vi "Start (App INI).vi"(7 "Splash Screen (Default)":refnum<class "Splash Screen.lvclass">, 8 "error in (no error)":errorcluster, 10 "INI Path (Default)":path) -> (0 "error out":errorcluster, 2 "MessageQ":refnum<class "MessageQ.lvclass">)   [LabVIEW 2020, in "Volatus.lvlib" / "Volatus Core.lvclass"]
uses:
  Volatus Core.lvclass
  MessageQ/MessageQ.lvclass
  Splash Screen/Splash Screen.lvclass
  Volatus Core.lvclass/Volatus Core.ctl
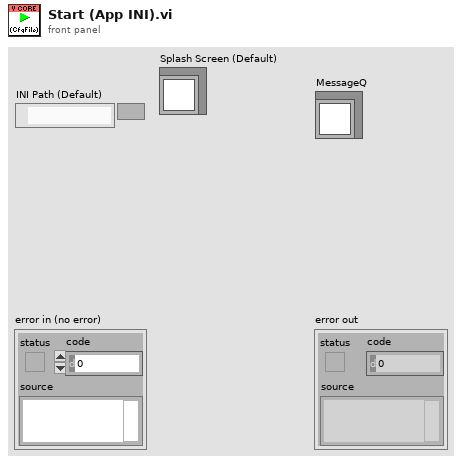
[diagram p1: front panel]
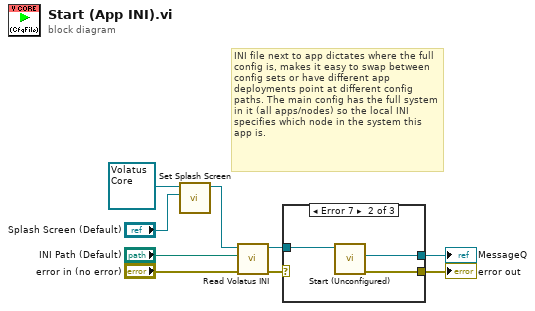
[diagram p0: block diagram]
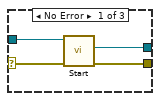
[diagram p2: hidden frame]
diagram:
  # "INI file next to app dictates where the full config is, makes it easy to swap between config sets or have different app deployments point at different config paths. The main config has the full system in it (all apps/nodes) so the local INI specifies which node in the system this app is."
  n1 = call "Set Splash Screen.vi"("Splash Screen"="Splash Screen (Default)", "Volatus Core in"=refnum<class "Volatus Core.lvclass"> refnum) -> ("Volatus Core out"=w1:refnum<class "Volatus Core.lvclass">)  [unwired: 8 in, 1 out]
  n2 = call "Read Volatus INI.vi"("error in (no error)"="error in (no error)", "INI Path (Default)"="INI Path (Default)", "Volatus Core in"=w1) -> ("error out"=w4:errorcluster, "Volatus Core out"=w5:refnum<class "Volatus Core.lvclass">)  [unwired: 7 in]
  n3 = case shown="Error 7" w4 {
    selector: w4 -> [w12 _ w17]
    tunnel: [w11 w15 w17] -> w7
    tunnel: [w10 w14 _] -> w8
    tunnel: w5 -> [w13 w16 _]
    frame No Error {
      n4 = call "Start.vi"("error in (no error)"=w12, "Volatus Core in"=w13) -> ("error out"=w11:errorcluster, "MessageQ"=w10:refnum<class "MessageQ.lvclass">)  [unwired: 8 in]
    }
    frame Error {
      n5 = call "Start (Unconfigured).vi"("Volatus Core in"=w16) -> ("error out"=w15:errorcluster, "MessageQ"=w14:refnum<class "MessageQ.lvclass">)  [unwired: 9 in]
    }
    frame Default {
    }
  }
  "error out" <- w7
  "MessageQ" <- w8
